vi "Func - FuncVI Refnums.vi"(5 "Params":T1, 6 "cmd (get)":T2(ring), 7 "Instance ID":u64 format="%.0x", 8 "error in":errorcluster, 11 "Func name":string) -> (0 "error out":errorcluster, 1 "loaded":bool, 2 "FuncVI RefNum out":refnum<vi>, 3 "FuncVI2 RefNum out":refnum<vi>, 4 "FuncVI2":bool)   [LabVIEW 2021]
doc: "::: CalcExpress Toolkit :::\nCopyright (c) 2000-2026 Konstantin Shifershteyn. All rights reserved."
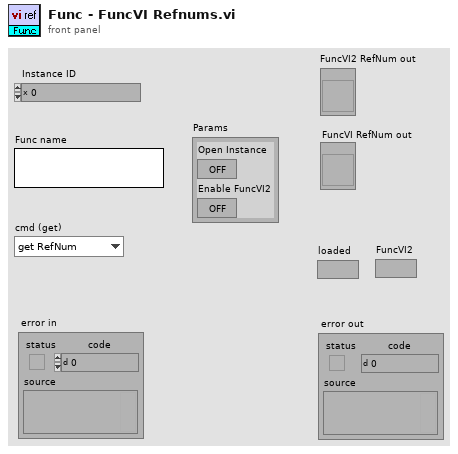
[diagram p1: front panel]
types:
  T1 = cluster{"Open Instance":bool, "Enable FuncVI2":bool}
  T2 = enum16{"get RefNum", "close Clones", "close RefNum", "close all RefNums", "update RefNums"}
  T3 = cluster{"FuncVI RefNum":refnum<vi>, "FuncVI2 RefNum":refnum<vi>}
  T4 = cluster{"Name":string, "Path":path, "Reentrant":bool, "FuncVI2":bool}
  T5 = cluster{"Name":string, "Path":path, "Reentrant":bool, "FuncVI2":bool}[]
  T6 = cluster{"FuncVI RefNum":refnum<vi>, "FuncVI2 RefNum":refnum<vi>}[]
  T7 = cluster{"FuncVI RefNum":bool, "FuncVI2 RefNum":bool}
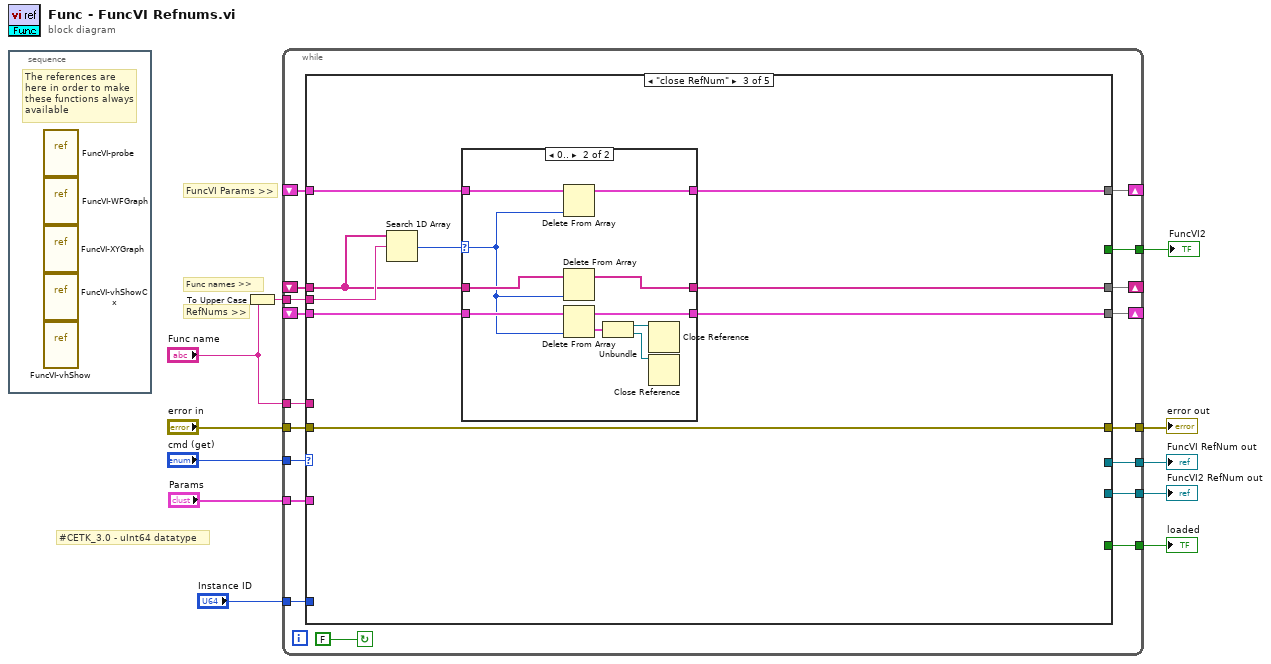
[diagram p0: block diagram]
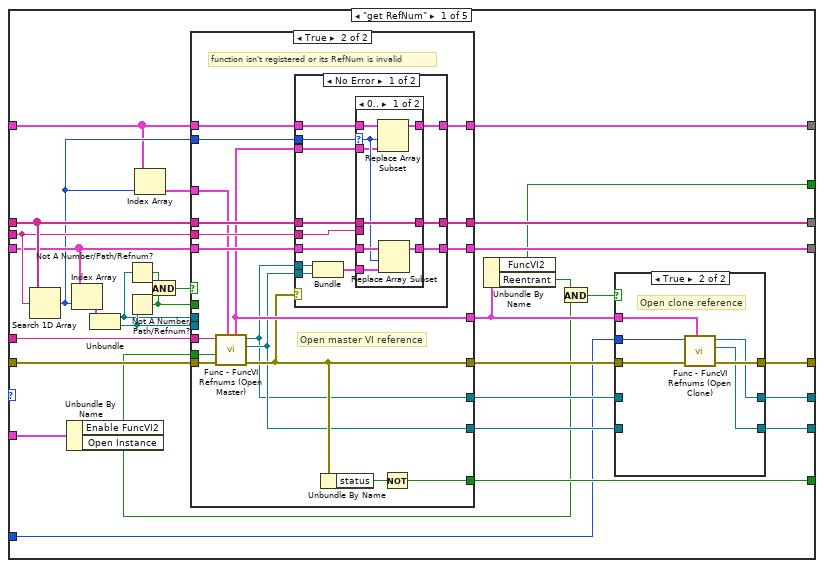
[diagram p2: hidden frame]
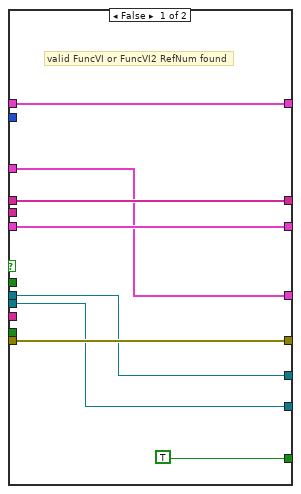
[diagram p4: hidden frame]
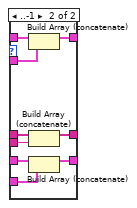
[diagram p5: hidden frame]
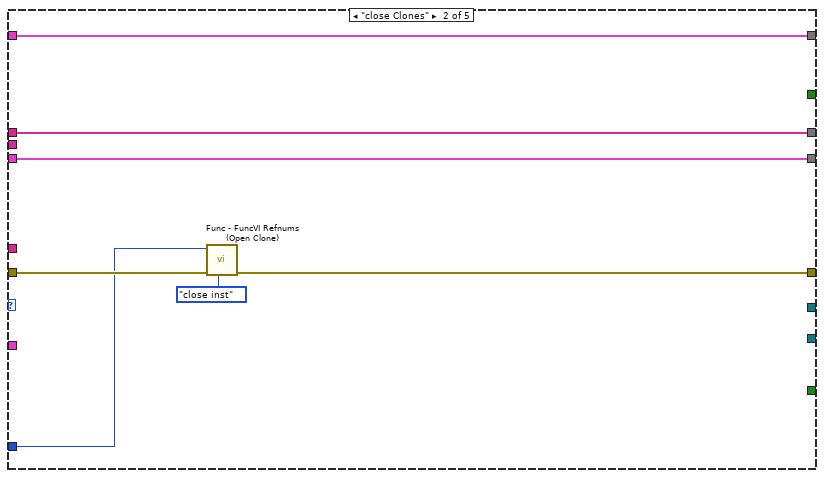
[diagram p7: hidden frame]
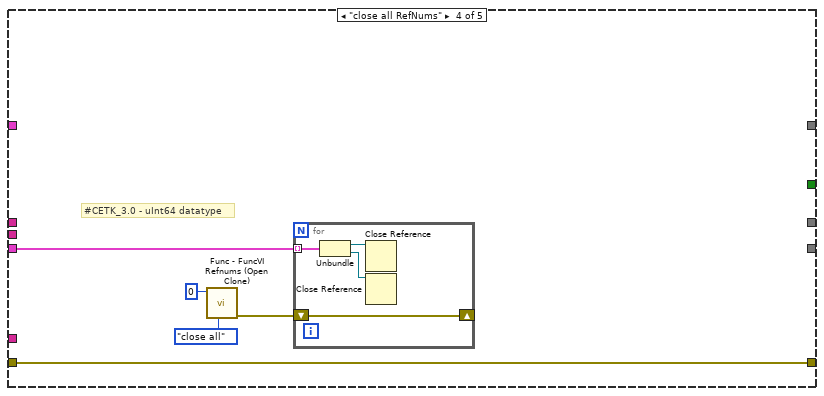
[diagram p9: hidden frame]
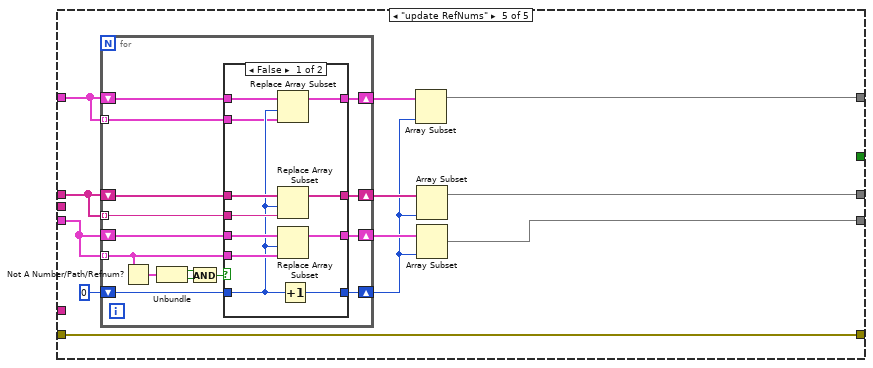
[diagram p10: hidden frame]
diagram:
  # "#CETK_3.0 - uInt64 datatype"
  # "RefNums >>"
  # "Func names >>"
  # "FuncVI Params >>"
  n1 = stacked-sequence {
    frame #0 {
      # "The references are\nhere in order to make\nthese functions always\navailable"
      n2 = vi-ref "FuncVI-probe.vi"() -> ()  [unwired: 1 out]
      n3 = vi-ref "FuncVI-WFGraph.vi"() -> ()  [unwired: 1 out]
      n4 = vi-ref "FuncVI-XYGraph.vi"() -> ()  [unwired: 1 out]
      n5 = vi-ref "FuncVI-vhShowCx.vi"() -> ()  [unwired: 1 out]
      n6 = vi-ref "FuncVI-vhShow.vi"() -> ()  [unwired: 1 out]
    }
  }
  n7 = To Upper Case(1:"Func name") -> (0:w7:string)
  n8 = while {
    tunnel: "Func name" -> [w19]
    tunnel: [w20] -> w6
    tunnel: "error in" -> [w21]
    tunnel: "cmd (get)" -> [w25]
    shift-left: _ -> [w23]
    shift-right: [w22] -> _
    shift-left: _ -> [w24]
    shift-right: [w27] -> _
    tunnel: [w28] -> w9
    tunnel: w7 -> [w26]
    tunnel: [w29] -> w11
    tunnel: [w17] -> w4
    shift-right: [w16] -> _
    shift-left: _ -> [w15]
    tunnel: [w14] -> w3
    tunnel: "Instance ID" -> [w13]
    tunnel: "Params" -> [w12]
    stop <- FALSE continue-if-true
    n9 = case shown="\"close RefNum\"" w25 {
      tunnel: [w42 w132 w139 w162 w172] -> w29
      tunnel: [w40 _ _ _ _] -> w28
      tunnel: [w61 w135 w140 _ w174] -> w27
      tunnel: w24 -> [w60 w135 w141 _ w171]
      tunnel: w26 -> [w59 _ w144 _ _]
      tunnel: w23 -> [w58 w134 w143 w161 w178]
      tunnel: [w57 w134 w142 _ w173] -> w22
      tunnel: w21 -> [w56 w131 w139 w162 w172]
      tunnel: [w55 _ _ _ _] -> w20
      tunnel: w19 -> [w54 _ _ _ _]
      tunnel: [w41 _ _ _ _] -> w17
      tunnel: [w47 w133 w137 _ w168] -> w16
      tunnel: w15 -> [w45 w133 w138 _ w167]
      tunnel: [w36 _ _ _ _] -> w14
      tunnel: w13 -> [w31 w130 _ _ _]
      tunnel: w12 -> [w30 _ _ _ _]
      frame "get RefNum" {
        n10 = Search 1D Array(1D array=w60, element=w59) -> (index of element=w46:i32)  [unwired: 1 in]
        n11 = Unbundle By Name(w30) -> ("Enable FuncVI2"=w33:bool, "Open Instance"=w32:bool)
        n12 = Index Array(array=w58, index=w46) -> (element=w53:T3)
        n13 = Unbundle(w53) -> ("FuncVI RefNum"=w51:refnum<vi>, "FuncVI2 RefNum"=w52:refnum<vi>)
        n14 = Not A Number/Path/Refnum?(number/path/refnum=w51) -> (NaN/Path/Refnum?=w50:bool)
        n15 = Not A Number/Path/Refnum?(number/path/refnum=w52) -> (NaN/Path/Refnum?=w48:bool)
        n16 = Index Array(array=w45, index=w46) -> (element=w44:T4)
        n17 = And(x=w50, y=w48) -> (x .and. y?=w49:bool)
        n18 = case shown="True" w49 {
          tunnel: [w75 w81] -> w43
          tunnel: w59 -> [_ w90]
          tunnel: w58 -> [w77 w96]
          tunnel: w60 -> [w78 w95]
          tunnel: [w78 w94] -> w61
          tunnel: [w77 w93] -> w57
          tunnel: w46 -> [_ w84]
          tunnel: w56 -> [w75 w92]
          tunnel: [TRUE w91] -> w55
          tunnel: w54 -> [_ w86]
          tunnel: w33 -> [_ w89]
          tunnel: w51 -> [w72 _]
          tunnel: w52 -> [w71 _]
          tunnel: w48 -> [_ _]
          tunnel: [w76 w87] -> w47
          tunnel: w45 -> [w76 w85]
          tunnel: w44 -> [w73 w83]
          tunnel: [w73 w82] -> w37
          tunnel: [w71 w80] -> w39
          tunnel: [w72 w79] -> w38
          frame False {
            # "valid FuncVI or FuncVI2 RefNum found"
          }
          frame True {
            # "Open master VI reference"
            # "function isn't registered or its RefNum is invalid"
            n19 = call "Func - FuncVI Refnums (Open Master).vi"("Func Info in"=w83, "error in"=w92, "open CSE FuncVI2 (F)"=w89, "Func name"=w86) -> ("error out"=w81:errorcluster, "FuncVI2 RefNum"=w80:refnum<vi>, "FuncVI RefNum"=w79:refnum<vi>, "Func Info out"=w82:T4)  [unwired: 4 in]
            n20 = case shown="No Error" w81 {
              tunnel: w96 -> [w104 w127]
              tunnel: w95 -> [w108 w128]
              tunnel: w79 -> [w102 _]
              tunnel: w90 -> [w107 _]
              tunnel: [w106 w128] -> w94
              tunnel: [w105 w127] -> w93
              tunnel: w84 -> [w103 _]
              tunnel: w80 -> [w101 _]
              tunnel: [w99 w126] -> w87
              tunnel: w85 -> [w98 w126]
              tunnel: w82 -> [w97 _]
              frame No Error {
                n21 = Bundle("FuncVI RefNum"=w102, "FuncVI2 RefNum"=w101) -> (w100:T3)  [unwired: 1 in]
                n22 = case shown="0.." w103 {
                  selector: w103 -> [w112 _]
                  tunnel: w104 -> [w113 w120]
                  tunnel: w108 -> [w116 w125]
                  tunnel: w100 -> [w114 w124]
                  tunnel: w107 -> [_ w123]
                  tunnel: [w116 w122] -> w106
                  tunnel: [w115 w121] -> w105
                  tunnel: [w111 w118] -> w99
                  tunnel: w98 -> [w110 w119]
                  tunnel: w97 -> [w109 w117]
                  frame 0.. {
                    n23 = Replace Array Subset(array=w110, new element=w109, index=w112) -> (w111:T5)
                    n24 = Replace Array Subset(array=w113, new element=w114, index=w112) -> (w115:T6)
                  }
                  frame ..-1 {
                    n25 = Build Array (concatenate)(w119, w117) -> (w118:T5)
                    n26 = Build Array (concatenate)(w125, w123) -> (w122:string[])
                    n27 = Build Array (concatenate)(w120, w124) -> (w121:T6)
                  }
                }
              }
              frame Error {
              }
            }
            n28 = Unbundle By Name(w81) -> ("status"=w88:bool)
            n29 = Not(x=w88) -> (.not. x?=w91:bool)
          }
        }
        n30 = Unbundle By Name(w37) -> ("FuncVI2"=w36:bool, "Reentrant"=w35:bool)
        n31 = And(x=w35, y=w32) -> (x .and. y?=w34:bool)
        n32 = case shown="True" w34 {
          tunnel: w43 -> [w64 w70]
          tunnel: [w64 w68] -> w42
          tunnel: [w63 w66] -> w41
          tunnel: [w62 w67] -> w40
          tunnel: w39 -> [w63 _]
          tunnel: w38 -> [w62 _]
          tunnel: w37 -> [_ w69]
          tunnel: w31 -> [_ w65]
          frame False {
          }
          frame True {
            # "Open clone reference"
            n33 = call "Func - FuncVI Refnums (Open Clone).vi"("Func Info in"=w69, "error in"=w70, "Instance ID"=w65) -> ("error out"=w68:errorcluster, "FuncVI2 RefNum"=w66:refnum<vi>, "FuncVI RefNum"=w67:refnum<vi>)  [unwired: 6 in]
          }
        }
      }
      frame "close Clones" {
        n34 = call "Func - FuncVI Refnums (Open Clone).vi"("cmd (get)"=enum16{"get", "close inst", "close all"}."close inst", "error in"=w131, "Instance ID"=w130) -> ("error out"=w132:errorcluster)  [unwired: 6 in, 2 out]
      }
      frame "close RefNum" {
        n35 = Search 1D Array(1D array=w141, element=w144) -> (index of element=w136:i32)  [unwired: 1 in]
        n36 = case shown="0.." w136 {
          selector: w136 -> [_ w148]
          tunnel: w143 -> [w147 w153]
          tunnel: [w147 w155] -> w142
          tunnel: w141 -> [w146 w157]
          tunnel: [w146 w156] -> w140
          tunnel: w138 -> [w145 w150]
          tunnel: [w145 w149] -> w137
          frame ..-1 {
          }
          frame 0.. {
            n37 = Delete From Array(array=w150, index=w148) -> (array with subset deleted=w149:T5)  [unwired: 1 in, 1 out]
            n38 = Delete From Array(array=w157, index=w148) -> (array with subset deleted=w156:string[])  [unwired: 1 in, 1 out]
            n39 = Delete From Array(array=w153, index=w148) -> (deleted portion=w154:T3, array with subset deleted=w155:T6)  [unwired: 1 in]
            n40 = Unbundle(w154) -> ("FuncVI RefNum"=w152:refnum<vi>, "FuncVI2 RefNum"=w151:refnum<vi>)
            n41 = Close Reference(reference=w152) -> ()  [unwired: 1 in, 1 out]
            n42 = Close Reference(reference=w151) -> ()  [unwired: 1 in, 1 out]
          }
        }
      }
      frame "close all RefNums" {
        # "#CETK_3.0 - uInt64 datatype"
        n43 = call "Func - FuncVI Refnums (Open Clone).vi"("cmd (get)"=enum16{"get", "close inst", "close all"}."close all", "Instance ID"=u64 0) -> ("error out"=w159:errorcluster)  [unwired: 7 in, 2 out]
        n44 = for {
          tunnel: w161 -> [w164] mode=indexing
          shift-right: [w163] -> _
          shift-left: w159 -> [w163]
          n45 = Unbundle(w164) -> ("FuncVI RefNum"=w166:refnum<vi>, "FuncVI2 RefNum"=w165:refnum<vi>)
          n46 = Close Reference(reference=w166) -> ()  [unwired: 1 in, 1 out]
          n47 = Close Reference(reference=w165) -> ()  [unwired: 1 in, 1 out]
        }
      }
      frame "update RefNums" {
        n48 = for {
          tunnel: w178 -> [w186] mode=indexing
          shift-right: [w191] -> w176
          shift-left: w171 -> [w193]
          shift-right: [w189] -> w175
          shift-left: w178 -> [w188]
          shift-right: [w190] -> w169
          shift-left: 0 -> [w192]
          tunnel: w171 -> [w185] mode=indexing
          shift-right: [w180] -> w170
          shift-left: w167 -> [w181]
          tunnel: w167 -> [w179] mode=indexing
          n49 = Not A Number/Path/Refnum?(number/path/refnum=w186) -> (NaN/Path/Refnum?=w187:T7)
          n50 = Unbundle(w187) -> ("FuncVI RefNum"=w184:bool, "FuncVI2 RefNum"=w183:bool)
          n51 = And(x=w184, y=w183) -> (x .and. y?=w182:bool)
          n52 = case shown="False" w182 {
            tunnel: w193 -> [w204 w208]
            tunnel: w192 -> [w197 w206]
            tunnel: [w203 w208] -> w191
            tunnel: [w202 w206] -> w190
            tunnel: w188 -> [w201 w207]
            tunnel: [w200 w207] -> w189
            tunnel: w186 -> [w199 _]
            tunnel: w185 -> [w198 _]
            tunnel: w181 -> [w196 w205]
            tunnel: [w195 w205] -> w180
            tunnel: w179 -> [w194 _]
            frame False {
              n53 = Replace Array Subset(array=w196, new element=w194, index=w197) -> (w195:T5)
              n54 = Replace Array Subset(array=w204, new element=w198, index=w197) -> (w203:string[])
              n55 = Replace Array Subset(array=w201, new element=w199, index=w197) -> (w200:T6)
              n56 = Increment(x=w197) -> (x+1=w202:i32)
            }
            frame True {
            }
          }
        }
        n57 = Array Subset(array=w170, length=w169) -> (w168:T5)  [unwired: 1 in]
        n58 = Array Subset(array=w176, length=w169) -> (w174:string[])  [unwired: 1 in]
        n59 = Array Subset(array=w175, length=w169) -> (w173:T6)  [unwired: 1 in]
      }
    }
  }
  "error out" <- w11
  "FuncVI RefNum out" <- w9
  "loaded" <- w6
  "FuncVI2 RefNum out" <- w4
  "FuncVI2" <- w3
